vi "Save Users File.vi"(4 "error in (no error)":errorcluster, 6 "Save":bool=TRUE, 7 "EasyUserManager in":refnum<class "EasyUserManager.lvclass">) -> (0 "error out":errorcluster, 3 "EasyUserManager out":refnum<class "EasyUserManager.lvclass">)   [LabVIEW 2024, in "EasyUserManager.lvclass"]
doc: "This VI increments the ChangeCount of the UsersFile and then, depending on the boolean input <B>Save</B>, saves the modified file without further prompt (Default: True). \n\nIf <B>Save</B> is False only the ChangeCount is incremented and you will see changes reflected through a * on the users file in teststand."
uses:
  EasyUserManager.lvclass
  EasyUserManager.lvclass/EasyUserManager.ctl
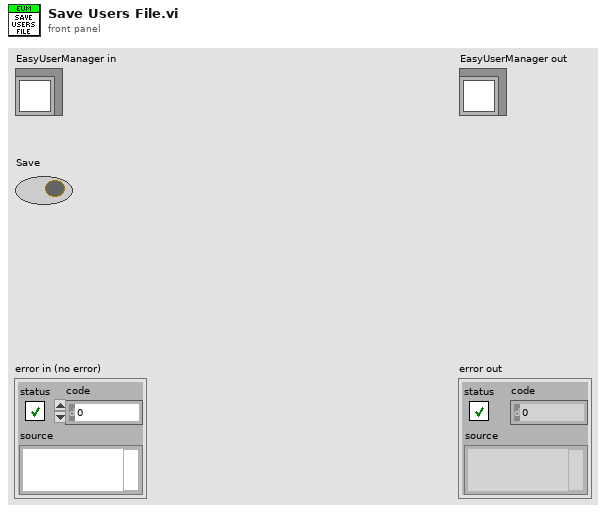
[diagram p1: front panel]
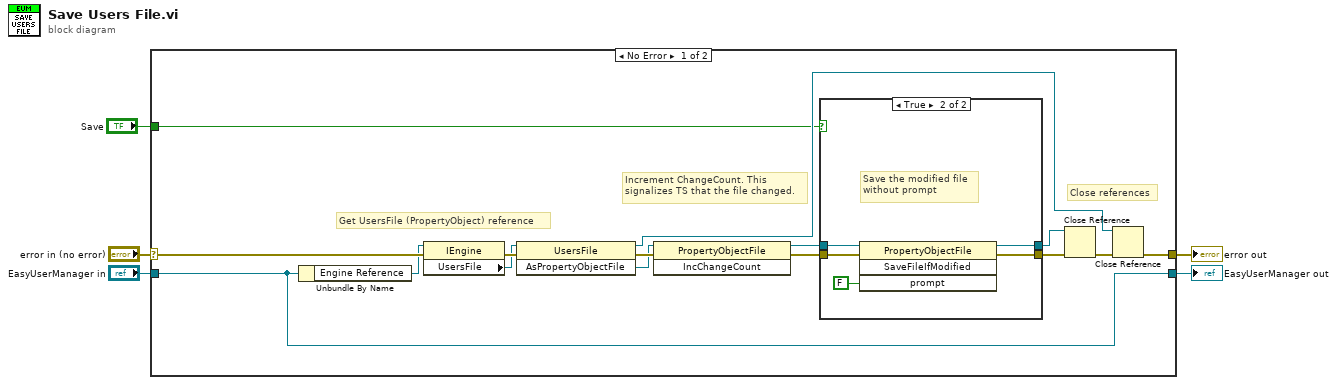
[diagram p0: block diagram]
diagram:
  n1 = case shown="No Error" "error in (no error)" {
    selector: "error in (no error)" -> [w19 w29]
    tunnel: [w20 w29] -> w4
    tunnel: [w18 w28] -> w2
    tunnel: "EasyUserManager in" -> [w18 w28]
    tunnel: "Save" -> [w6 _]
    frame No Error {
      # "Close references"
      # "Increment ChangeCount. This\nsignalizes TS that the file changed."
      # "Get UsersFile (PropertyObject) reference"
      n2 = Unbundle By Name(w18) -> ("Engine Reference"=w7:refnum<k7>)
      n3 = property on="Property Node" class="IEngine"(reference=w7, error in=w19) -> (error out=w10:errorcluster, "UsersFile"=w8:refnum<k7>)  [unwired: 1 out]
      n4 = invoke on="Invoke Node" class="UsersFile" method="AsPropertyObjectFile"(reference=w8, error in=w10) -> (reference out=w12:refnum<k7>, error out=w11:errorcluster, "AsPropertyObjectFile"=w9:refnum<k7>)  [unwired: 1 in]
      n5 = invoke on="Invoke Node" class="PropertyObjectFile" method="IncChangeCount"(reference=w9, error in=w11) -> (reference out=w14:refnum<k7>, error out=w15:errorcluster)  [unwired: 1 in, 1 out]
      n6 = case shown="True" w6 {
        tunnel: [w21 w27] -> w17
        tunnel: [w22 w26] -> w16
        tunnel: w15 -> [w21 w25]
        tunnel: w14 -> [w22 w24]
        frame False {
        }
        frame True {
          # "Save the modified file\nwithout prompt"
          n7 = invoke on="Invoke Node" class="PropertyObjectFile" method="SaveFileIfModified"(reference=w24, error in=w25, "prompt"=FALSE) -> (reference out=w26:refnum<k7>, error out=w27:errorcluster)  [unwired: 1 in, 2 out]
        }
      }
      n8 = Close Reference(reference=w16, error in (no error)=w17) -> (error out=w13:errorcluster)
      n9 = Close Reference(reference=w12, error in (no error)=w13) -> (error out=w20:errorcluster)
    }
    frame Error {
      # "Pass error and do nothing."
    }
  }
  "error out" <- w4
  "EasyUserManager out" <- w2
